vi "CreateCompatibleDC Wrapper Template.vi"(0 "hdc":u64, 11 "error in":errorcluster) -> (4 "HDC":u64, 15 "error out":errorcluster)   [LabVIEW 2020]
doc: "Creates a memory device context compatible with hdc through gdi32.dll CreateCompatibleDC (stdcall, called in any thread). Delete it with gdi32 DeleteDC.vi. When error in carries an error the DLL is not called. Generated by scripts\\Build Win32 Wrappers.vi - do not edit by hand, rebuild it."
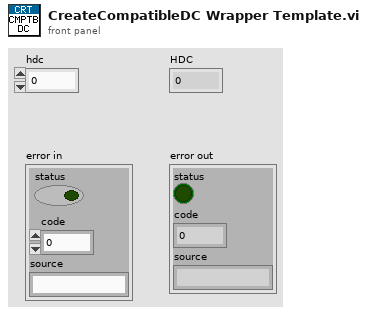
[diagram p1: front panel]
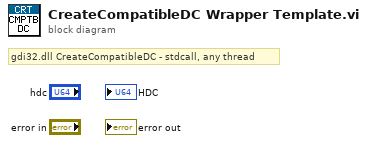
[diagram p0: block diagram]
diagram:
  # "gdi32.dll CreateCompatibleDC - stdcall, any thread"
